vi "X-Axis_Step.vi"(9 "Left?":bool, 10 "X Motor":refnum<k7>) -> ()   [LabVIEW 2024]
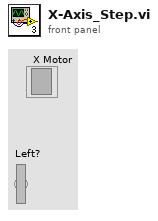
[diagram p1: front panel]
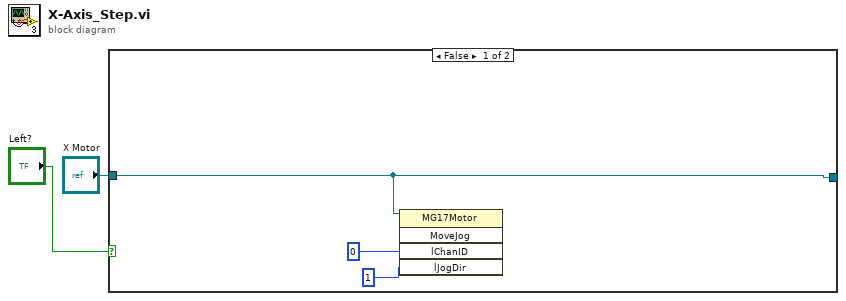
[diagram p0: block diagram]
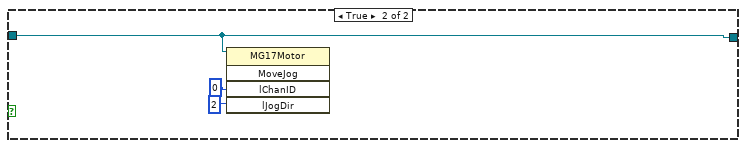
[diagram p2: hidden frame]
diagram:
  n1 = case shown="False" "Left?" {
    tunnel: "X Motor" -> [w3 w6]
    tunnel: [w3 w6] -> _
    frame False {
      n2 = invoke class="MG17Motor" method="MoveJog"(reference=w3, "lChanID"=0, "lJogDir"=1) -> ()  [unwired: 2 in, 5 out]
    }
    frame True {
      n3 = invoke class="MG17Motor" method="MoveJog"(reference=w6, "lChanID"=0, "lJogDir"=2) -> ()  [unwired: 2 in, 5 out]
    }
  }
